vi "J1939_Signal_Validator.vi"() -> ()   [LabVIEW 2026]
panel:
  in  "lower limit":dbl
  in  "upper limit":dbl=3000.0
  in  "Offset":dbl=256.0 format="%#_13g"
  in  "Scaling":dbl=0.125
  in  "EEC1 Payload":u8[](array[numeric])
  out "Engine Speed (RPM)":dbl
  out "Validation Result":string
  out "Signal Valid?":bool
  # "J1939 EEC1 Engine Speed Validator\nEnter an 8-byte EEC1 payload (PGN 61444) in decimal and click Run. The VI decodes bytes 4 and 5 into engine speed (SPN 190). The Signal Valid? LED turns on when the payload contains exactly 8 bytes and the decoded RPM is within the configured limits."
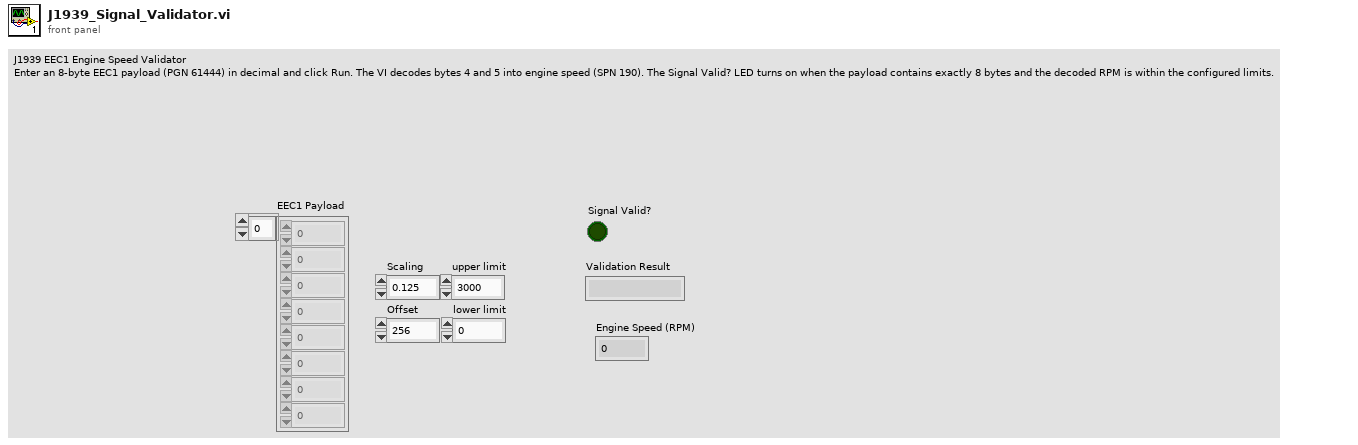
[diagram p1: front panel]
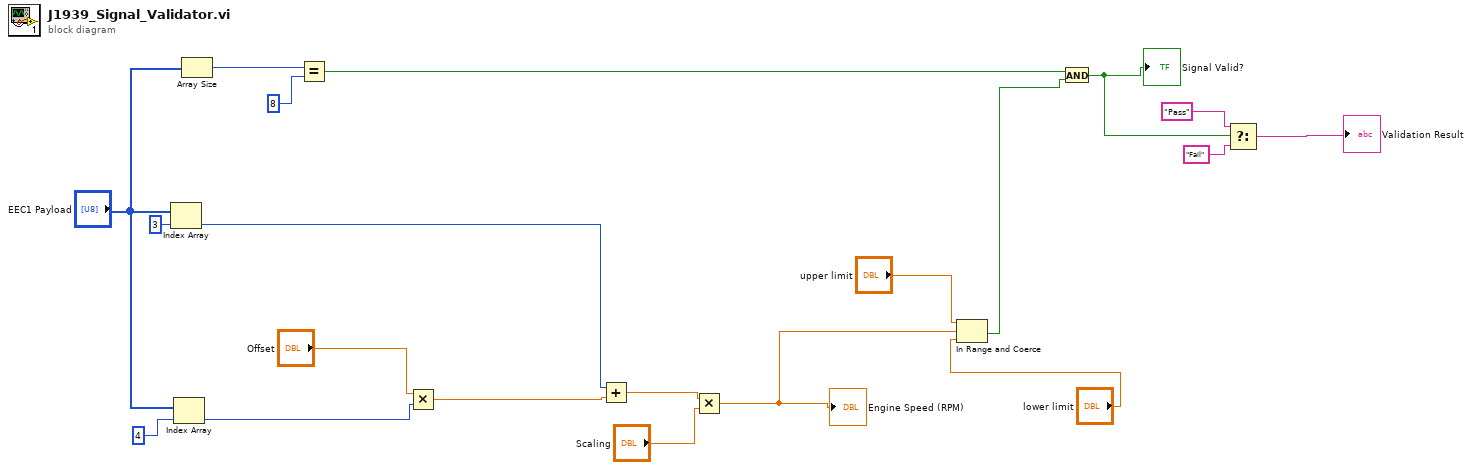
[diagram p0: block diagram]
diagram:
  n1 = Index Array(array="EEC1 Payload", index=3) -> (element=w11:u8)
  n2 = Index Array(array="EEC1 Payload", index=4) -> (element=w10:u8)
  n3 = Array Size(array="EEC1 Payload") -> (size(s)=w9:i32)
  n4 = Equal?(x=w9, y=8) -> (x = y?=w7:bool)
  n5 = Multiply(x="Offset", y=w10) -> (x*y=w15:dbl)
  n6 = Add(x=w11, y=w15) -> (x+y=w14:dbl)
  n7 = Multiply(x=w14, y="Scaling") -> (x*y=w17:dbl)
  "Engine Speed (RPM)" <- w17
  n8 = In Range and Coerce(upper limit="upper limit", x=w17, lower limit="lower limit") -> (In Range?=w5:bool)  [unwired: 1 out]
  n9 = And(x=w7, y=w5) -> (x .and. y?=w4:bool)
  "Signal Valid?" <- w4
  n10 = Select(t="Pass", s=w4, f="Fail") -> (s? t:f=→"Validation Result":string)
